vi "Update Operation Typedef.vi"(9 "VI Refs":refnum<vi>[](array[refnum]), 10 "Imm Cmd String":string, 11 "Subsysten Name":string) -> (1 "VI Refs":refnum<vi>[](array[refnum]), 3 "Imm Cmds":string[](array[string]))   [LabVIEW 2023]
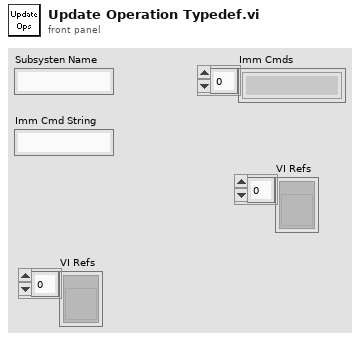
[diagram p1: front panel]
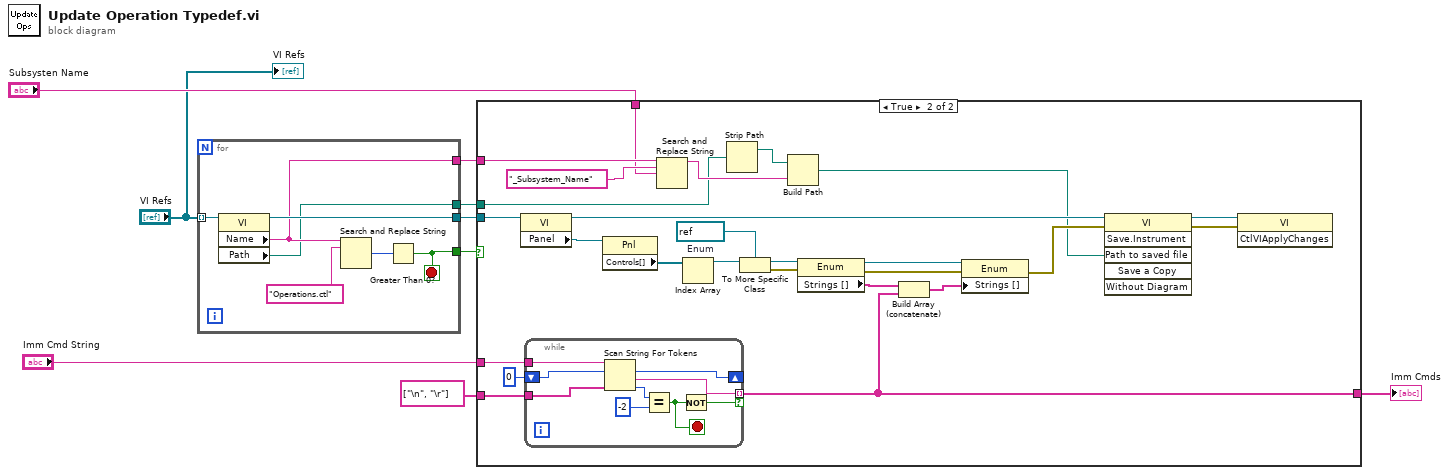
[diagram p0: block diagram]
diagram:
  n1 = for {
    tunnel: "VI Refs" -> [w14] mode=indexing
    tunnel: [w10] -> w2
    tunnel: [w13] -> w3
    tunnel: [w12] -> w6
    tunnel: [w11] -> w8
    stop <- w10 stop-if-true
    n2 = property class="VI"(reference=w14) -> (reference out=w13:refnum<vi>, "Name"=w12:string, "Path"=w11:path)  [unwired: 1 in, 1 out]
    n3 = Search and Replace String(input string=w12, search string="Operations.ctl") -> (number of replacements=w15:i32)  [unwired: 6 in, 3 out]
    n4 = Greater Than 0?(x=w15) -> (x > 0?=w10:bool)
  }
  n5 = case shown="True" w2 {
    tunnel: w3 -> [_ w42]
    tunnel: "Imm Cmd String" -> [_ w33]
    tunnel: string[] ["\n", "\r"] ("delimiters (\\s,\\t,\\r,\\n)") -> [_ w17]
    tunnel: w6 -> [_ w27]
    tunnel: "Subsysten Name" -> [_ w25]
    tunnel: w8 -> [_ w23]
    tunnel: [_ w18] -> w9
    frame False {
    }
    frame True {
      w38 = refnum<vi> refnum  # Enum
      n6 = property class="VI"(reference=w42) -> (reference out=w28:refnum<vi>, "Panel"=w41:refnum<vi>)  [unwired: 1 in, 1 out]
      n7 = while {
        tunnel: w33 -> [w51]
        shift-right: [w49] -> _
        shift-left: 0 ("y") -> [w50]
        tunnel: w17 -> [w48]
        tunnel: [w47] -> w18 mode=indexing if=w43
        stop <- w44 stop-if-true
        n8 = Scan String For Tokens(6:w48, 8:w50, 9:w51) -> (0:w46:i32, 1:w47:string, 2:w49:i32)  [unwired: 3 in, 1 out]
        n9 = Equal?(x=w46, y=-2) -> (x = y?=w44:bool)
        n10 = Not(x=w44) -> (.not. x?=w43:bool)
      }
      n11 = property class="Pnl"(reference=w41) -> ("Controls[]"=w40:refnum<vi>[])  [unwired: 1 in, 2 out]
      n12 = Search and Replace String(input string=w27, search string="_Subsystem_Name", replace string=w25) -> (result string=w24:string)  [unwired: 5 in, 3 out]
      n13 = Index Array(array=w40) -> (element=w39:refnum<vi>)  [unwired: 1 in]
      n14 = Strip Path(path=w23) -> (stripped path=w22:path)  [unwired: 1 out]
      n15 = To More Specific Class(target class=w38, reference=w39) -> (specific class reference=w37:refnum<vi>, error out=w36:errorcluster)  [unwired: 1 in]
      n16 = Build Path(base path=w22, name or relative path=w24) -> (appended path=w21:path)
      n17 = property class="Enum"(reference=w37, error in=w36) -> (reference out=w35:refnum<vi>, error out=w34:errorcluster, "Strings []"=w31:string[])
      n18 = Build Array (concatenate)(w31, w18) -> (w30:string[])
      n19 = property class="Enum"(reference=w35, error in=w34, "Strings []"=w30) -> (error out=w29:errorcluster)  [unwired: 1 out]
      n20 = invoke class="VI" method="Save.Instrument"(reference=w28, error in=w29, "Path to saved file"=w21) -> (reference out=w20:refnum<vi>, error out=w19:errorcluster)  [unwired: 3 in, 4 out]
      n21 = invoke class="VI" method="CtlVIApplyChanges"(reference=w20, error in=w19) -> ()  [unwired: 1 in, 3 out]
    }
  }
  "Imm Cmds" <- w9
  "VI Refs" <- "VI Refs"
